vi "CO reference TurnTable.vi"(8 "error in (no error)":errorcluster caption="에러 입력(에러 없음)", 11 "Instrument Manager 입력":refnum<class "Instrument Manager.lvclass">) -> (0 "error out":errorcluster caption="에러 출력", 3 "Instrument Manager 출력":refnum<class "Instrument Manager.lvclass">)   [LabVIEW 2023, in "Instrument Manager.lvclass"]
uses:
  Instrument Manager.lvclass
  Module/Turn Table and Mast Control/Class/CO3000/CO3000.lvclass
  Module/Turn Table and Mast Control/Interface Class/Turn Table/Interface - Turn Table.lvclass
  Instrument Manager.lvclass/Instrument Manager.ctl
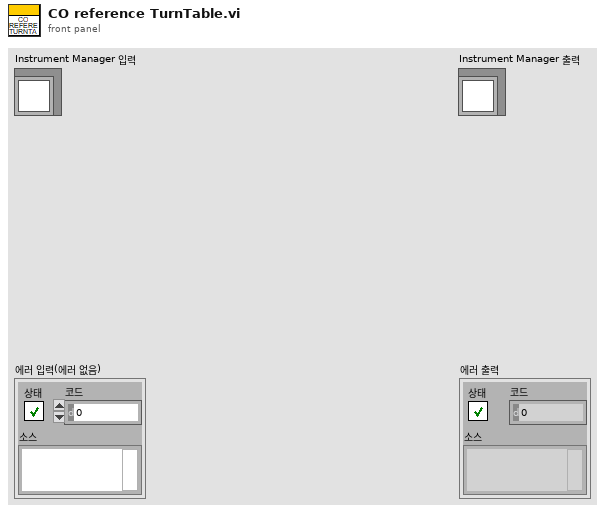
[diagram p1: front panel]
types:
  T1 = cluster{"Anritsu Call Box":refnum<class "Anritsu Call Box.lvclass">, "Spectrum Analyzer":refnum<class "Interface_Spectrum.lvclass">, "RF Switch Box":refnum<class "RF Filter Box.lvclass">, "Turn Table":refnum<class "Interface - Turn Table.lvclass">, "Mast":refnum<class "Interface - Mast.lvclass">, "3D Controller":refnum<class "Interface_3D Controller.lvclass">}
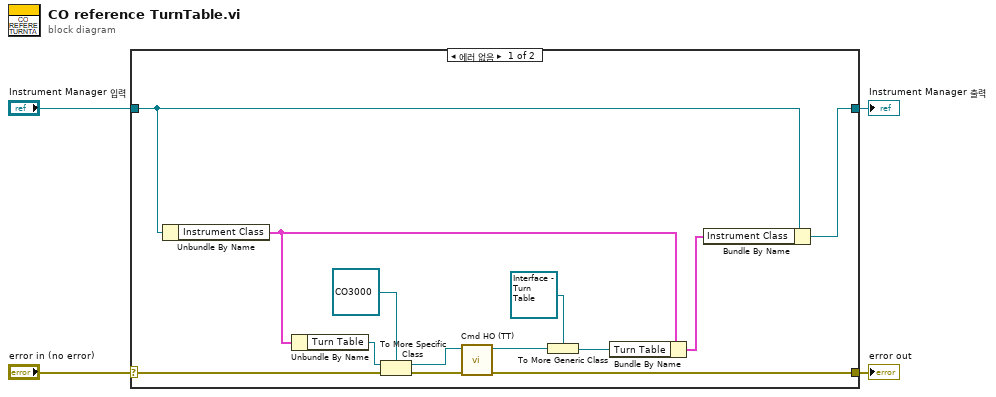
[diagram p0: block diagram]
diagram:
  n1 = case shown="에러 없음" "error in (no error)" {
    selector: "error in (no error)" -> [w15 w19]
    tunnel: [w5 w19] -> w3
    tunnel: [w6 w18] -> w1
    tunnel: "Instrument Manager 입력" -> [w17 w18]
    frame No Error {
      n2 = Unbundle By Name(w17) -> ("Instrument Class"=w10:T1)
      n3 = Unbundle By Name(w10) -> ("Turn Table"=w16:refnum<class "Interface - Turn Table.lvclass">)
      n4 = To More Specific Class(target class=refnum<class "CO3000.lvclass"> refnum ("Turn Table and Mast.lvlib:CO3000.lvclass"), reference=w16, error in=w15) -> (specific class reference=w13:refnum<class "CO3000.lvclass">, error out=w12:errorcluster)
      n5 = call-dynamic "Cmd HO (TT).vi"("error in (no error)"=w12, "CO3000 입력"=w13) -> ("error out"=w5:errorcluster, "CO3000 출력"=w11:refnum<class "CO3000.lvclass">)  [unwired: 8 in]
      n6 = To More Generic Class(target class=refnum<class "Interface - Turn Table.lvclass"> refnum ("Turn Table and Mast.lvlib:Interface - Turn Table.lvclass"), reference=w11) -> (generic class reference=w8:refnum<class "Interface - Turn Table.lvclass">)
      n7 = Bundle By Name(cluster=w10, "Turn Table"=w8) -> (w7:T1)
      n8 = Bundle By Name(cluster=w17, "Instrument Class"=w7) -> (w6:refnum<class "Instrument Manager.lvclass">)
    }
    frame Error {
    }
  }
  "error out" <- w3
  "Instrument Manager 출력" <- w1
